vi "clone.vi"(0 "reference":refnum<class "ClassNode.lvclass">, 5 "error in (no error)":errorcluster) -> (14 "reference out":refnum<class "ClassNode.lvclass">, 15 "clonedClassNode":refnum<class "AbstractNode.lvclass">, 19 "error out":errorcluster)   [LabVIEW 2020, in "ClassNode.lvclass"]
doc: "public Object clone()"
uses:
  <resource>/Framework/Providers/Open_GDS/UML/ClassNode_class/ClassNode.lvclass
  C:/Program Files (x86)/National Instruments/LabVIEW 2020/resource/Framework/Providers/Open_GDS/UML/RectangularNode_class/RectangularNode.lvclass
  C:/Program Files (x86)/National Instruments/LabVIEW 2020/resource/Framework/Providers/Open_GDS/UML/AbstractNode_class/AbstractNode.lvclass
  <resource>/Framework/Providers/Open_GDS/UML/AbstractNode_class/AbstractNode.lvclass
  <resource>/Framework/Providers/Open_GDS/UML/MultiLineString_class/MultiLineString.lvclass
  <resource>/Framework/Providers/Open_GDS/UML/RectangularNode_class/RectangularNode.lvclass
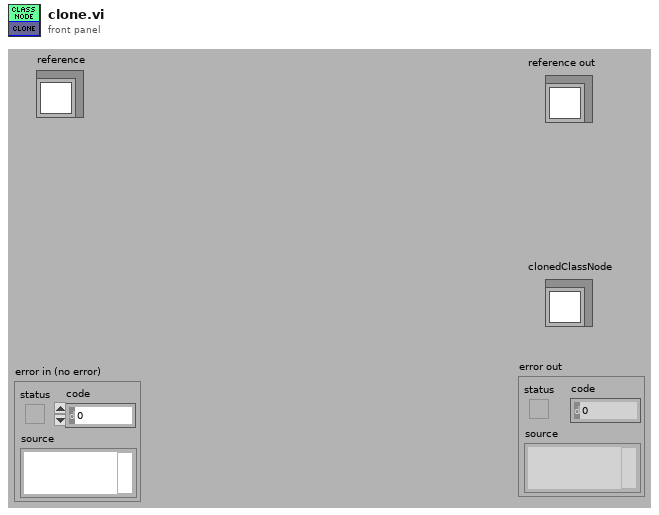
[diagram p1: front panel]
types:
  T1 = typedef "ClassNode.lvclass/ObjectAttributes.ctl" = cluster{"midHeight":dbl, "botHeight":dbl, "name":refnum<class "MultiLineString.lvclass">, "attributes":refnum<class "MultiLineString.lvclass">, "methods":refnum<class "MultiLineString.lvclass">, "DEFAULT_COMPARTMENT_HEIGHT":i32, "DEFAULT_WIDTH":i32, "DEFAULT_HEIGHT":i32, "showMethods":bool, "showAttributes":bool, "ClassPath":path}
  T2 = typedef "RectangularNode.lvclass/ObjectAttributes.ctl" = cluster{"bounds":T3}
  T3 = typedef "Rectangle Rectangle2D.ctl" = cluster{"x":dbl, "y":dbl, "width":dbl, "height":dbl}
  T4 = typedef "AbstractNode.lvclass/ObjectAttributes.ctl" = cluster{"parent":refnum<class "AbstractNode.lvclass">, "children":refnum<class "AbstractNode.lvclass">[], "Hidden":bool}
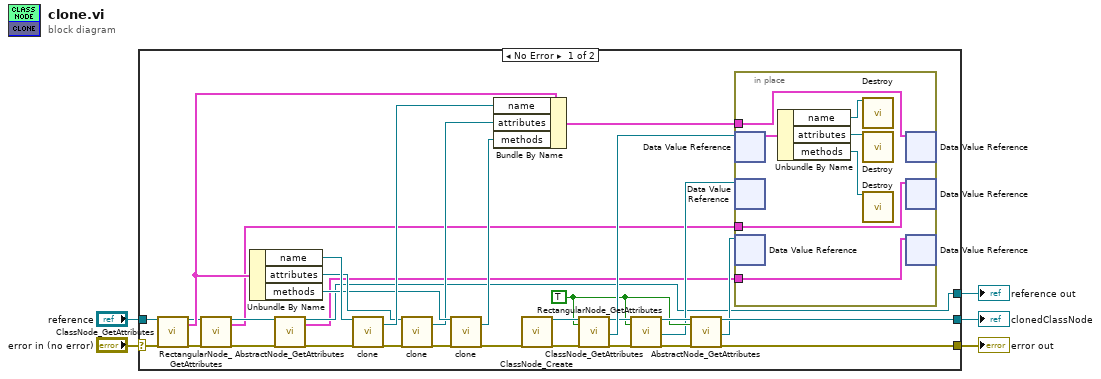
[diagram p0: block diagram]
diagram:
  n1 = case shown="No Error" "error in (no error)" {
    selector: "error in (no error)" -> [w37 w46]
    tunnel: "reference" -> [w38 w47]
    tunnel: [w17 w46] -> w4
    tunnel: [w8 w47] -> w3
    tunnel: [w19 _] -> w1
    frame No Error {
      w16 = TRUE ("OnlyGetDvrReference(False)")
      n2 = call <resource>:"ClassNode_GetAttributes.vi"("reference in"=w38, "error in (no error)"=w37) -> ("reference out"=w9:refnum<class "ClassNode.lvclass">, "Data"=w25:T1, "error out"=w13:errorcluster)  [unwired: 1 in, 14 out]
      n3 = call <resource>:"RectangularNode_GetAttributes.vi"("reference in"=w9, "error in (no error)"=w13) -> ("reference out"=w12:refnum<class "ClassNode.lvclass">, "Data"=w7:T2, "error out"=w11:errorcluster)  [unwired: 14 in, 1 out]
      n4 = Unbundle By Name(w25) -> ("name"=w36:refnum<class "MultiLineString.lvclass">, "attributes"=w32:refnum<class "MultiLineString.lvclass">, "methods"=w31:refnum<class "MultiLineString.lvclass">)
      n5 = call <resource>:"AbstractNode_GetAttributes.vi"("reference in"=w12, "error in (no error)"=w11) -> ("reference out"=w8:refnum<class "ClassNode.lvclass">, "Data"=w6:T4, "error out"=w10:errorcluster)  [unwired: 14 in, 1 out]
      n6 = call-dynamic "clone.vi"("reference"=w36, "error in (no error)"=w10) -> ("clonedMultiLineString"=w35:refnum<class "MultiLineString.lvclass">, "error out"=w34:errorcluster)  [unwired: 15 in, 1 out]
      n7 = call-dynamic "clone.vi"("reference"=w32, "error in (no error)"=w34) -> ("clonedMultiLineString"=w30:refnum<class "MultiLineString.lvclass">, "error out"=w33:errorcluster)  [unwired: 15 in, 1 out]
      n8 = call-dynamic "clone.vi"("reference"=w31, "error in (no error)"=w33) -> ("clonedMultiLineString"=w29:refnum<class "MultiLineString.lvclass">, "error out"=w26:errorcluster)  [unwired: 15 in, 1 out]
      n9 = Bundle By Name(cluster=w25, "name"=w35, "attributes"=w30, "methods"=w29) -> (w23:T1)
      n10 = call <resource>:"ClassNode_Create.vi"("error in (no error)"=w26) -> ("reference out"=w28:refnum<class "ClassNode.lvclass">, "error out"=w27:errorcluster)  [unwired: 17 in]
      n11 = call <resource>:"ClassNode_GetAttributes.vi"("reference in"=w28, "OnlyGetDvrReference(False)"=w16, "error in (no error)"=w27) -> ("reference out"=w20:refnum<class "ClassNode.lvclass">, "DataRef"=w24:refnum<data-value>, "error out"=w22:errorcluster)  [unwired: 13 in, 1 out]
      n12 = call <resource>:"RectangularNode_GetAttributes.vi"("reference in"=w20, "OnlyGetDvrReference(False)"=w16, "error in (no error)"=w22) -> ("reference out"=w21:refnum<class "ClassNode.lvclass">, "DataRef"=w14:refnum<data-value>, "error out"=w18:errorcluster)  [unwired: 13 in, 1 out]
      n13 = call <resource>:"AbstractNode_GetAttributes.vi"("reference in"=w21, "OnlyGetDvrReference(False)"=w16, "error in (no error)"=w18) -> ("reference out"=w19:refnum<class "ClassNode.lvclass">, "DataRef"=w15:refnum<data-value>, "error out"=w17:errorcluster)  [unwired: 13 in, 1 out]
      n14 = in-place {
        in-place-border: w23 -> [w45]
        in-place-border: w7 -> [w40]
        in-place-border: w6 -> [w39]
        n15 = in-place-dvr #1(w24) -> (w44:T1)  [unwired: 1 out]
        n16 = in-place-dvr #2(w14) -> ()  [unwired: 2 out]
        n17 = in-place-dvr #3(w15) -> ()  [unwired: 2 out]
        n18 = Unbundle By Name(w44) -> ("name"=w43:refnum<class "MultiLineString.lvclass">, "attributes"=w42:refnum<class "MultiLineString.lvclass">, "methods"=w41:refnum<class "MultiLineString.lvclass">)
        n19 = call-dynamic "Destroy.vi"("reference"=w43) -> ()  [unwired: 17 in, 2 out]
        n20 = call-dynamic "Destroy.vi"("reference"=w42) -> ()  [unwired: 17 in, 2 out]
        n21 = call-dynamic "Destroy.vi"("reference"=w41) -> ()  [unwired: 17 in, 2 out]
        n22 = in-place-dvr #1(w45) -> ()  [unwired: 2 out]
        n23 = in-place-dvr #2(w40) -> ()  [unwired: 2 out]
        n24 = in-place-dvr #3(w39) -> ()  [unwired: 2 out]
      }
    }
    frame Error {
    }
  }
  "reference out" <- w3
  "error out" <- w4
  "clonedClassNode" <- w1
